vi "search passw&permission.vi"(8 "error in (no error)":errorcluster caption="错误输入（无错误）", 10 "索引":i32=2, 11 "数组":string[][](array[string])) -> (0 "error out":errorcluster caption="错误输出", 3 "元素":string)   [LabVIEW 2018, in "login.lvlib"]
uses:
  login.lvlib
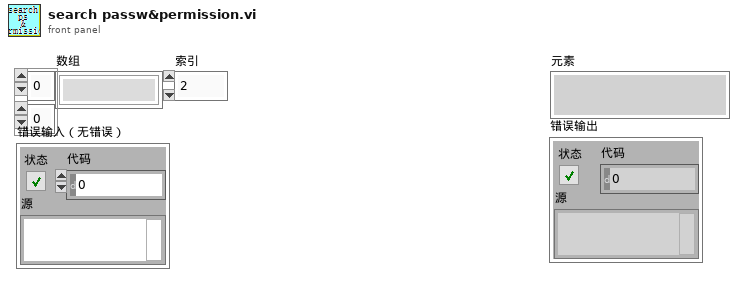
[diagram p1: front panel]
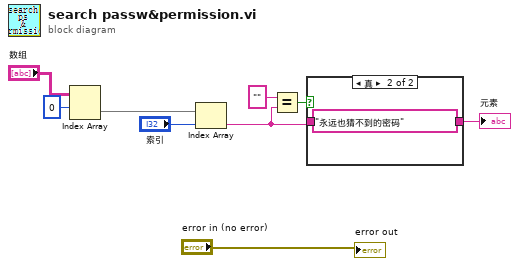
[diagram p0: block diagram]
diagram:
  n1 = Index Array(array="数组", index (row)=0 ("索引")) -> (element=w9:string[])  [unwired: 1 in]
  n2 = Index Array(array=w9, index="索引") -> (element=w1:string)
  n3 = Equal?(x="", y=w1) -> (x = y?=w3:bool)
  n4 = case shown="真" w3 {
    tunnel: [w10 "永远也猜不到的密码"] -> w2
    tunnel: w1 -> [w10 _]
    frame False {
    }
    frame True {
    }
  }
  "元素" <- w2
  "error out" <- "error in (no error)"
